vi "Free FPGA String.vi"(8 "error in (no error)":errorcluster caption="错误输入（无错误）", 11 "strFPGA":string) -> (0 "error out":errorcluster caption="错误输出", 3 "strFPGA out":string)   [LabVIEW 2017, in "smncsftmt.lvlib"]
doc: "__declspec(dllexport) void FreeFPGAString(char* strFPGA);"
uses:
  smncsftmt.lvlib
  smncsftmt.dll
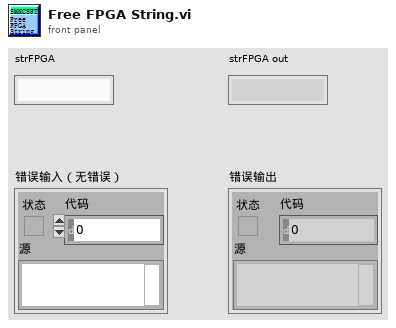
[diagram p1: front panel]
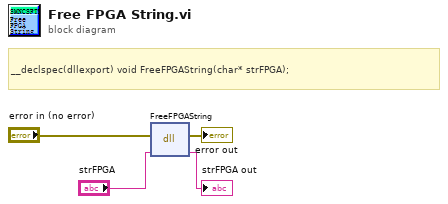
[diagram p0: block diagram]
diagram:
  # "__declspec(dllexport) void FreeFPGAString(char* strFPGA);"
  n1 = dll-call lib="PTH2oabs CUsersaDesktop\nLABVIEW范例National InstrumentsLabVIEW 2017user.lib\tsmncsftmtsmncsftmt.*" fn="FreeFPGAString"(error in="error in (no error)", "strFPGA"="strFPGA") -> (error out=→"error out":errorcluster, "strFPGA"=→"strFPGA out":string)  [unwired: 3 in, 1 out]
